vi "Validate HTTP Request.vi"(6 "protocol version exists":bool, 7 "origin exists":bool, 8 "error in":errorcluster, 9 "protocol version":string, 10 "method":string, 11 "origin":string) -> (0 "error out":errorcluster, 1 "payload":string, 2 "status code":u16, 3 "accepted?":bool)   [LabVIEW 2020, in "MCP Server.lvlib"]
doc: "Decides whether an incoming HTTP request may be handed to the MCP request handler, following the MCP Streamable HTTP transport rules. Pure decision logic with scalar terminals and no side effects.\n\nChecks, in this order:\n1. method must be exactly POST, otherwise status 405.\n2. Origin (DNS rebinding protection): an absent header is accepted. A present one must be http or https followed by localhost, 127.0.0.1 or [::1] with an optional numeric port, compared case-insensitively. Anything else, including the literal null, gives status 403.\n3. MCP-Protocol-Version: an absent header is accepted. A present one must be one of all versions in Supported Protocol Versions.vi, modern or legacy (checked by Is Supported Protocol Version.vi), otherwise status 400.\n\nWhen accepted? is TRUE, status code is 200 and payload is empty. When it is FALSE, status code is 405, 403 or 400 and payload is a JSON-RPC error object (id null) to be sent with Content-Type application/json: code -32600 for 405 and 403, and for 400 the MCP 2026-07-28 error -32022 Unsupported protocol version with data.supported and data.requested (Build Unsupported Version Error.vi), in both eras, so that dual-era clients recognise a modern server.\n\nThe modern-era checks of the other headers (Mcp-Method, Mcp-Name, MCP-Protocol-Version against params._meta) need the body and are made by Handle MCP Request.vi.\n\nThe error cluster is passed through unchanged. The decision is computed regardless of error in."
uses:
  MCP Server.lvlib
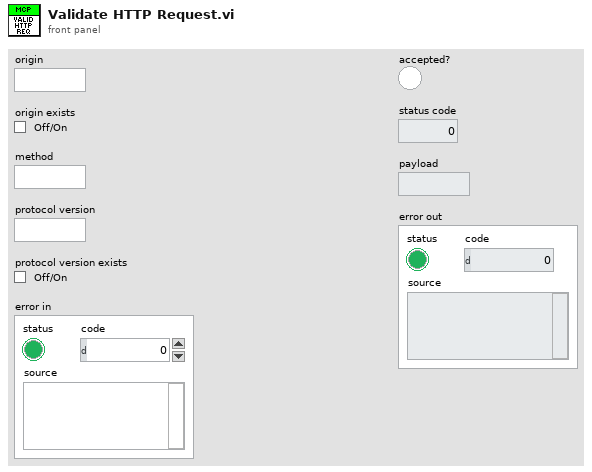
[diagram p1: front panel]
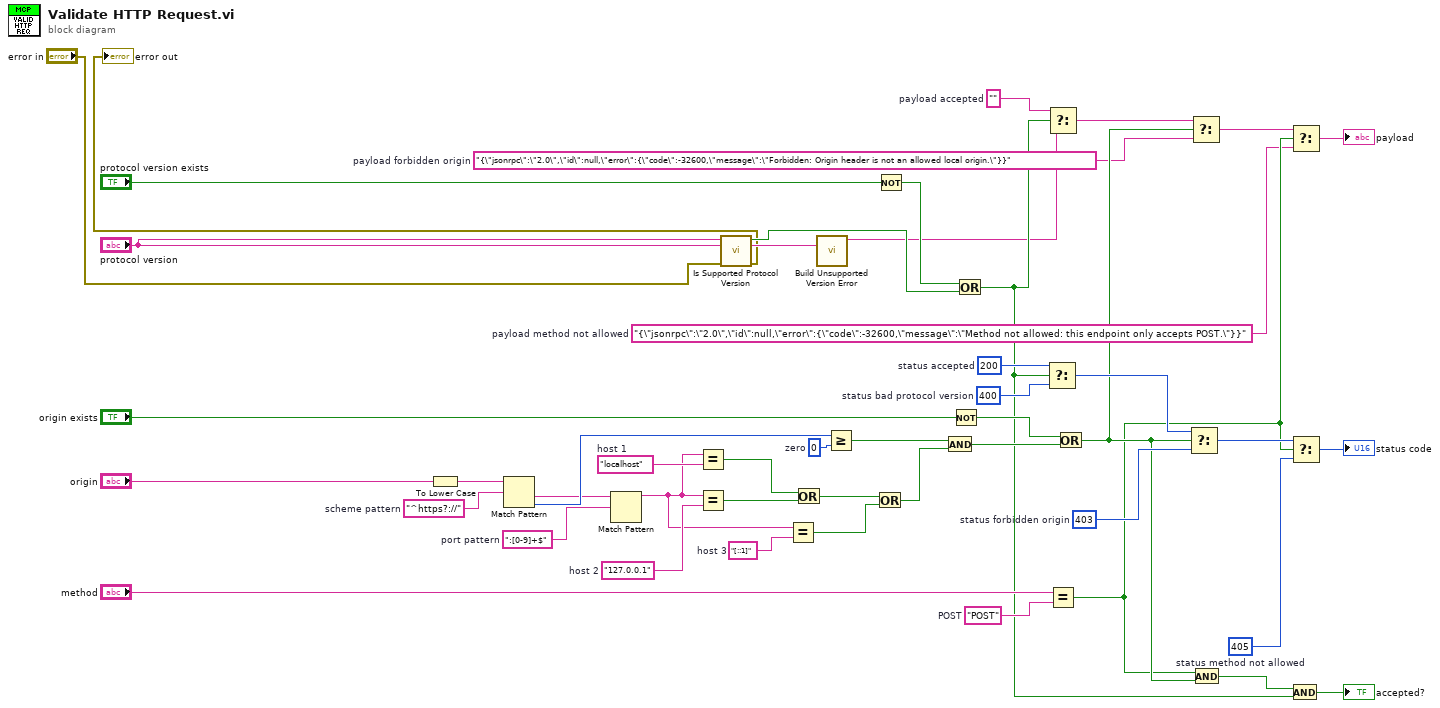
[diagram p0: block diagram]
diagram:
  w8 = "{\"jsonrpc\":\"2.0\",\"id\":null,\"error\":{\"code\":-32600,\"message\":\"Method not allowed: this endpoint only accepts POST.\"}}"  # payload method not allowed
  w11 = "{\"jsonrpc\":\"2.0\",\"id\":null,\"error\":{\"code\":-32600,\"message\":\"Forbidden: Origin header is not an allowed local origin.\"}}"  # payload forbidden origin
  w15 = ""  # payload accepted
  w16 = u16 405  # status method not allowed
  w18 = u16 403  # status forbidden origin
  w20 = u16 400  # status bad protocol version
  w21 = u16 200  # status accepted
  w35 = "[::1]"  # host 3
  w37 = "127.0.0.1"  # host 2
  w38 = "localhost"  # host 1
  w39 = ":[0-9]+$"  # port pattern
  w41 = 0  # zero
  w43 = "^https?://"  # scheme pattern
  w46 = "POST"  # POST
  n1 = To Lower Case(string="origin") -> (all lower case string=w44:string)
  n2 = Match Pattern(string=w44, regular expression=w43) -> (after substring=w40:string, offset past match=w42:i32)  [unwired: 1 in, 2 out]
  n3 = Match Pattern(string=w40, regular expression=w39) -> (before substring=w36:string)  [unwired: 1 in, 3 out]
  n4 = Equal?(x=w36, y=w38) -> (x = y?=w34:bool)
  n5 = Equal?(x=w36, y=w37) -> (x = y?=w33:bool)
  n6 = call "Is Supported Protocol Version.vi"("error in"="error in", "protocol version"="protocol version") -> ("error out"=→"error out":errorcluster, "supported?"=w4:bool)  [unwired: 8 in]
  n7 = Equal?(x=w36, y=w35) -> (x = y?=w31:bool)
  n8 = Or(x=w34, y=w33) -> (x .or. y?=w32:bool)
  n9 = call "Build Unsupported Version Error.vi"("requested version"="protocol version") -> ("payload"=w1:string)  [unwired: 9 in, 1 out]
  n10 = Greater Or Equal?(x=w42, y=w41) -> (x >= y?=w30:bool)
  n11 = Or(x=w32, y=w31) -> (x .or. y?=w29:bool)
  n12 = Not(x="protocol version exists") -> (.not. x?=w23:bool)
  n13 = And(x=w30, y=w29) -> (x .and. y?=w26:bool)
  n14 = Not(x="origin exists") -> (.not. x?=w27:bool)
  n15 = Or(x=w23, y=w4) -> (x .or. y?=w14:bool)
  n16 = Select(t=w21, s=w14, f=w20) -> (s? t:f=w19:u16)
  n17 = Select(t=w15, s=w14, f=w1) -> (s? t:f=w13:string)
  n18 = Equal?(x="method", y=w46) -> (x = y?=w9:bool)
  n19 = Or(x=w27, y=w26) -> (x .or. y?=w12:bool)
  n20 = Select(t=w19, s=w12, f=w18) -> (s? t:f=w17:u16)
  n21 = Select(t=w13, s=w12, f=w11) -> (s? t:f=w10:string)
  n22 = And(x=w9, y=w12) -> (x .and. y?=w22:bool)
  n23 = And(x=w22, y=w14) -> (x .and. y?=→"accepted?":bool)
  n24 = Select(t=w10, s=w9, f=w8) -> (s? t:f=→"payload":string)
  n25 = Select(t=w17, s=w9, f=w16) -> (s? t:f=→"status code":u16)
